vi "Initialize with Switch Parameters Core.vi"(8 "error in (no error)":errorcluster, 10 "Switch Parameters in":refnum<class "Abstract Switch Init Parameters.lvclass">, 11 "Mock NI-SWITCH Consumer in":refnum<class "Mock NI-SWITCH Consumer.lvclass">=refnum) -> (0 "error out":errorcluster, 3 "Mock NI-SWITCH Consumer out":refnum<class "Mock NI-SWITCH Consumer.lvclass">)   [LabVIEW 2020, in "Mock NI-SWITCH Consumer.lvclass"]
uses:
  Mock NI-SWITCH Consumer.lvclass
  Includes/CDMessaging.lvlibp/Switch/Abstract Switch Init Parameters/Abstract Switch Init Parameters.lvclass
  Mock NI-SWITCH Consumer.lvclass/Mock NI-SWITCH Consumer.ctl
  NI-SWITCH Consumer/NI-SWITCH Consumer.lvclass
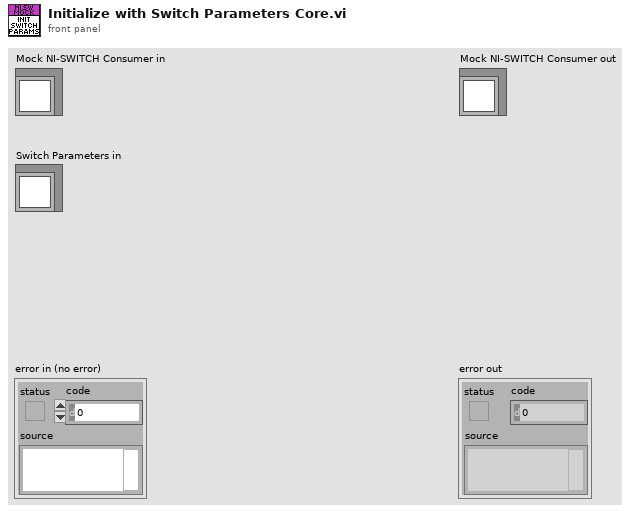
[diagram p1: front panel]
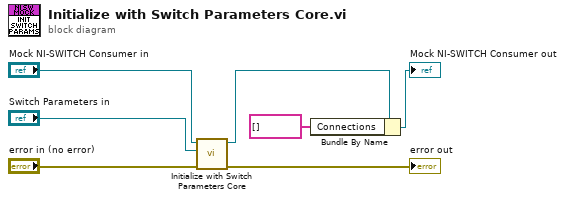
[diagram p0: block diagram]
diagram:
  n1 = call-parent "Initialize with Switch Parameters Core.vi"("error in (no error)"="error in (no error)", "Switch Parameters in"="Switch Parameters in", "NI-SWITCH Consumer in"="Mock NI-SWITCH Consumer in") -> ("error out"=→"error out":errorcluster, "NI-SWITCH Consumer out"=w3:refnum<class "Mock NI-SWITCH Consumer.lvclass">)  [unwired: 7 in]
  n2 = Bundle By Name(cluster=w3, "Connections"=string[] []) -> (→"Mock NI-SWITCH Consumer out":refnum<class "Mock NI-SWITCH Consumer.lvclass">)
